vi "Write Dig Chx.vi"(4 "Line":string(combo)="/Line0", 6 "Port":string(combo)="/Port0", 8 "error in":errorcluster, 9 "Device":string, 10 "Ch Value":bool) -> (0 "error out":errorcluster)   [LabVIEW 2013]
uses:
  <vilib>/DAQmx/write.llb/DAQmx Write.vi
  <vilib>/DAQmx/write.llb/DAQmx Write (Digital 1D Bool NChan 1Samp 1Line).vi
  <vilib>/DAQmx/create/channels.llb/DAQmx Create Channel (DO-Digital Output).vi
  <vilib>/DAQmx/miscellaneous.llb/DAQmx Fill In Error Info.vi
  <resource>/objmgr/daqmx.rc
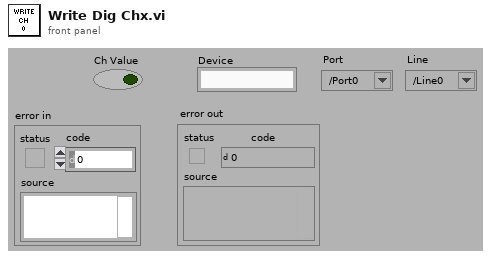
[diagram p1: front panel]
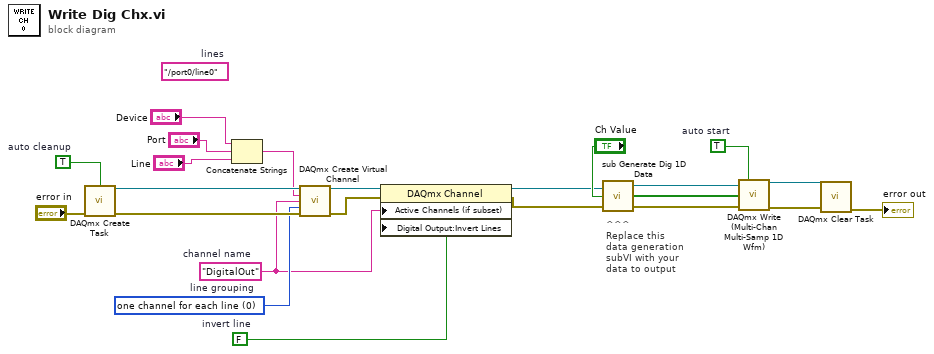
[diagram p0: block diagram]
diagram:
  (unwired) "/port0/line0"  # lines
  w11 = FALSE  # invert line
  w14 = 0 items=["one channel for each line", "one channel for all lines"]  # line grouping
  w8 = "DigitalOut"  # channel name
  w16 = TRUE  # auto cleanup
  w23 = TRUE  # auto start
  # "^^^\nReplace this\ndata generation\nsubVI with your\ndata to output"
  n1 = call <vilib>:"DAQmx Create Task.vi"("auto cleanup"=w16, "error in"="error in") -> ("task out"=w15:refnum<k21>, "error out"=w17:errorcluster)  [unwired: 12 in]
  n2 = Concatenate Strings("Device", "Port", "Line") -> (w1:string)
  n3 = call-poly <vilib>:"DAQmx Create Virtual Channel.vi"("task in"=w15, "lines"=w1, "name to assign"=w8, "line grouping"=w14, "error in"=w17) -> ("task out"=w13:refnum<k21>, "error out"=w12:errorcluster)  [unwired: 9 in]
  n4 = property class="DAQmx Channel"(reference=w13, error in=w12, "Active Channels (if subset)"=w8, "Digital Output:Invert Lines"=w11) -> (reference out=w9:refnum<k21>, error out=w10:errorcluster)
  n5 = call <vilib>:"sub Generate Dig 1D Data.vi"("error in"=w10, "initial value"="Ch Value", "task in"=w9) -> ("error out"=w21:errorcluster, "Data"=w20:bool[], "task out"=w19:refnum<k21>)
  n6 = call-poly "DAQmx Write (Multi-Chan Multi-Samp 1D Wfm).vi"("task/channels in"=w19, "auto start"=w23, "data"=w20, "error in"=w21) -> ("task out"=w6:refnum<k21>, "error out"=w7:errorcluster)  [unwired: 9 in, 1 out]
  n7 = call <vilib>:"DAQmx Clear Task.vi"("task in"=w6, "error in"=w7) -> ("error out"=→"error out":errorcluster)  [unwired: 13 in]
